vi "PGPASS.Write.vi"(8 "error in":errorcluster, 11 "Connections":T1[](array[typedef])) -> (0 "error out":errorcluster)   [LabVIEW 2019, in "PGPASS.lvlib"]
uses:
  PGPASS.lvlib
  PGPASS.Connection Information.ctl
  3f3501ec-8c9a-41d7-90ce-62519d153c74.vi
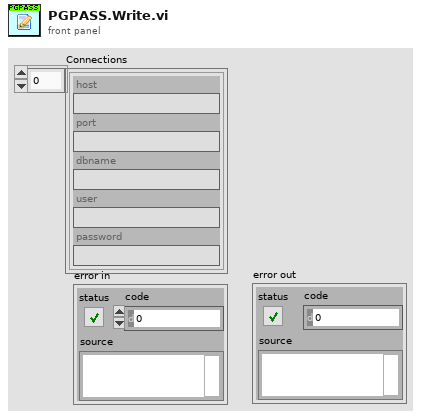
[diagram p1: front panel]
types:
  T1 = typedef "PGPASS.lvlib/PGPASS.Connection Information.ctl" = cluster{"host":string, "port":string, "dbname":string, "user":string, "password":string}
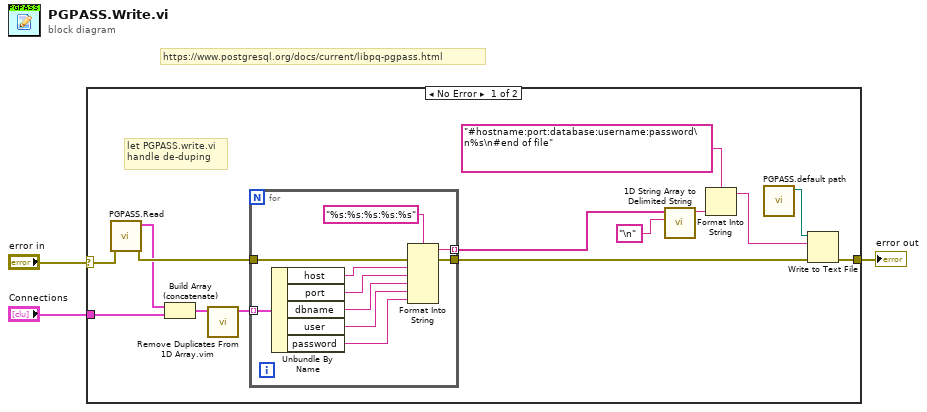
[diagram p0: block diagram]
diagram:
  # "https://www.postgresql.org/docs/current/libpq-pgpass.html"
  n1 = case shown="No Error" "error in" {
    selector: "error in" -> [w9 w28]
    tunnel: [w17 w28] -> w3
    tunnel: "Connections" -> [w5 _]
    frame No Error {
      # "let PGPASS.write.vi\nhandle de-duping"
      n2 = call "PGPASS.Read.vi"("error in"=w9) -> ("error out"=w8:errorcluster, "Connections"=w7:T1[])  [unwired: 9 in]
      n3 = Build Array (concatenate)(w7, w5) -> (w6:T1[])
      n4 = call "Remove Duplicates From 1D Array.vim"("array"=w6) -> ("array with duplicates removed"=w4:T1[])  [unwired: 10 in]
      n5 = for {
        tunnel: [w26] -> w10 mode=indexing
        tunnel: w4 -> [w25] mode=indexing
        tunnel: [w22] -> w16
        tunnel: w8 -> [w18]
        n6 = Unbundle By Name(w25) -> ("host"=w20:string, "port"=w21:string, "dbname"=w23:string, "user"=w24:string, "password"=w19:string)
        n7 = Format Into String(format string="%s:%s:%s:%s:%s", error in=w18, w20, w21, w23, w24, w19) -> (resulting string=w26:string, error out=w22:errorcluster)  [unwired: 1 in]
      }
      n8 = call <vilib>:"1D String Array to Delimited String.vi"("delimiter"="\n", "string array"=w10) -> ("delimited string"=w13:string)  [unwired: 9 in]
      n9 = Format Into String(format string="#hostname:port:database:username:password\n%s\n#end of file", w13) -> (resulting string=w12:string)  [unwired: 2 in, 1 out]
      n10 = call "PGPASS.default path.vi"() -> ("PGPASS path"=w15:path)  [unwired: 10 in, 1 out]
      n11 = Write to Text File(file (use dialog)=w15, text=w12, error in=w16) -> (error out=w17:errorcluster)  [unwired: 1 in, 2 out]
    }
    frame Error {
    }
  }
  "error out" <- w3
